vi "Event Handler.vi"(0 "uService Template in":refnum<class "Dummy.lvclass">, 5 "Event type":T1=enum."Message", 7 "Item Name":string, 9 "Data":variant, 11 "error in (no error)":errorcluster) -> (4 "uService Template out":refnum<class "Dummy.lvclass">, 15 "error out":errorcluster)   [LabVIEW 2020, in "Dummy.lvlib" / "Dummy.lvclass"]
doc: "This VI is the event handler of the uService: every time an event is triggered to the uService, this VI is called.\nNote: here you can access the Actor/Class data, but it will be the one coming out from Init. You cannot modify the values.\nThree different events are supported:\nI) Button Pressed: get called on a GUI button pressed. Item Name is the name (label) of the button, Data is empty.\nII) Shared Variable Updated: get called when a SV you subscribed to is updated. Item Name is the name of the SV, and Data is the value (note: you need to convert it to the proper type).\nIII) Message: get called every time a user event is generated using Send Message to Event Handler. The values of Item Name and Data are the one given to the Send Message to Event Handler.\nIV) Ready to launch?: this frame get called every time a new Run is initiated. Each uService is responsible of performing a self check before giving back the green light for the Run to start."
uses:
  Dummy.lvclass
  Dummy.lvclass/Dummy.ctl
  TALOS/TALOS_PPL.lvlibp/Father of all uServices/Father of all uServices/Father of all uServices.lvclass
  C:/LabVIEW Code/aegis-labview-code/TALOS/TALOS_PPL.lvlibp/Father of all uServices/Father of all uServices/Father of all uServices.lvclass
  TALOS/TALOS_PPL.lvlibp/Father of all uServices/Father of all uServices/Event Handler Items.ctl
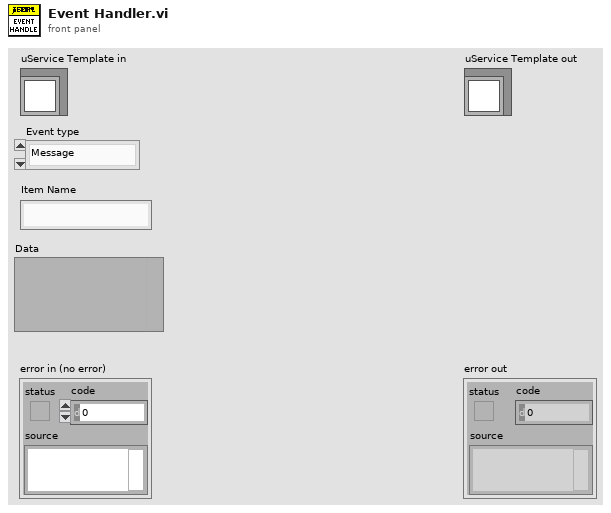
[diagram p1: front panel]
types:
  T1 = typedef "TALOS_PPL.lvlibp/Father of all uServices.lvlib/Father of all uServices.lvclass/Event Handler Items.ctl" = enum16{"Button Pressed", "Message", "Ready to launch?", "Safe Mode", "Start RUN", "Stop RUN"}
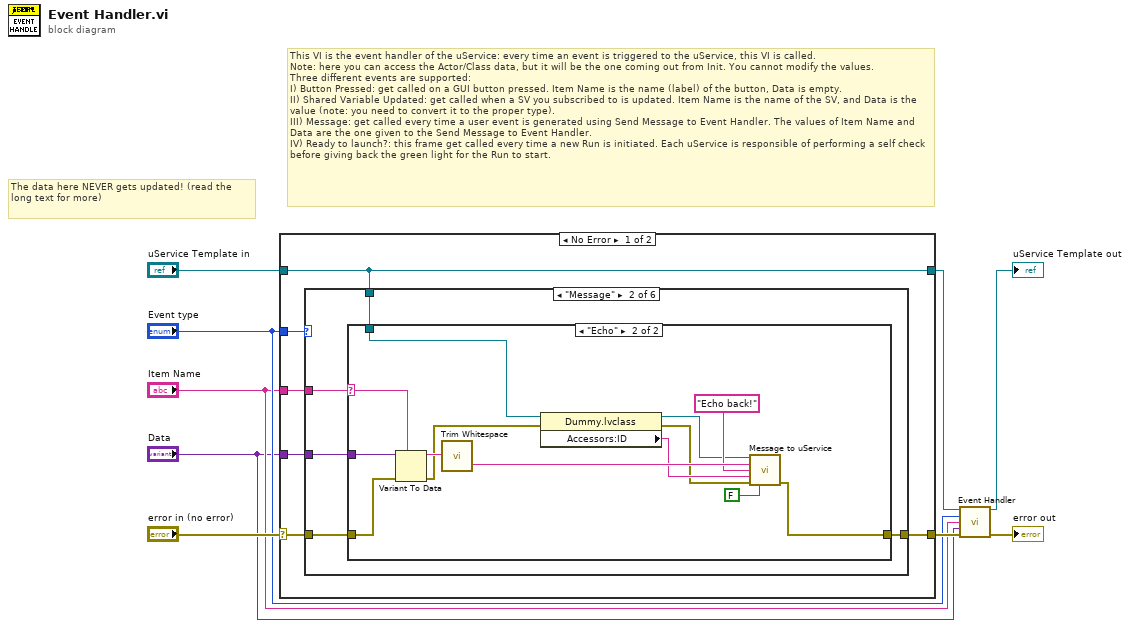
[diagram p0: block diagram]
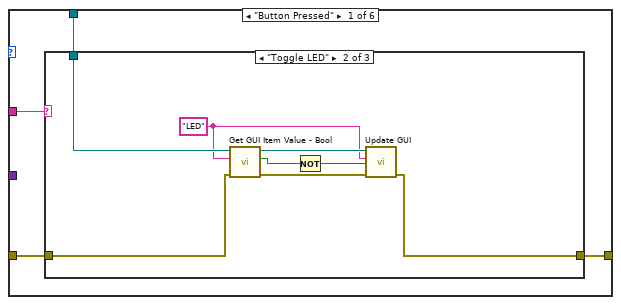
[diagram p2: hidden frame]
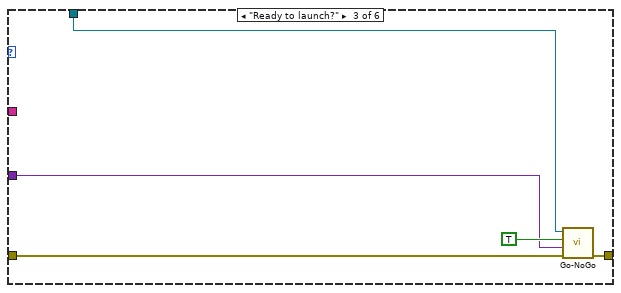
[diagram p6: hidden frame]
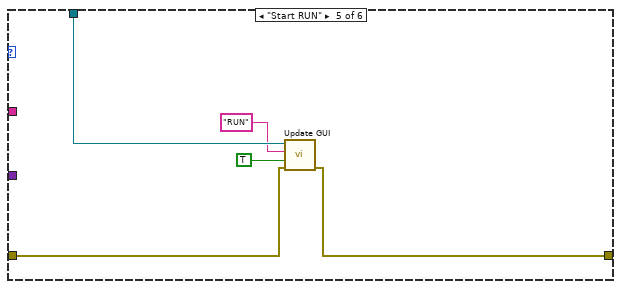
[diagram p8: hidden frame]
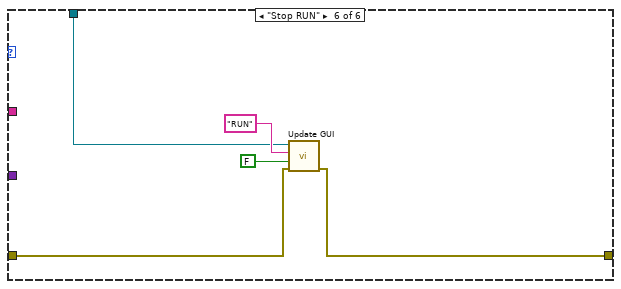
[diagram p9: hidden frame]
diagram:
  # "The data here NEVER gets updated! (read the long text for more)"
  # "This VI is the event handler of the uService: every time an event is triggered to the uService, this VI is called.\nNote: here you can access the Actor/Class data, but it will be the one coming out from Init. You cannot modify the values.\nThree different events are supported:\nI) Button Pressed: get called on a GUI button pressed. Item Name is the name (label) of the button, Data is empty.\nII) Shared Variable Updated: get called when a SV you subscribed to is updated. Item Name is the name of the SV, and Data is the value (note: you need to convert it to the proper type).\nIII) Message: get called every time a user event is generated using Send Message to Event Handler. The values of Item Name and Data are the one given to the Send Message to Event Handler.\nIV) Ready to launch?: this frame get called every time a new Run is initiated. Each uService is responsible of performing a self check before giving back the green light for the Run to start."
  n1 = case shown="No Error" "error in (no error)" {
    selector: "error in (no error)" -> [w13 w66]
    tunnel: [w14 w66] -> w7
    tunnel: [w12 w65] -> w4
    tunnel: "uService Template in" -> [w12 w65]
    tunnel: "Event type" -> [w15 _]
    tunnel: "Item Name" -> [w11 _]
    tunnel: "Data" -> [w10 _]
    frame No Error {
      n2 = case shown="\"Message\"" w15 {
        tunnel: [w19 w30 w52 w54 w56 w61] -> w14
        tunnel: w13 -> [w16 w34 w53 w54 w55 w60]
        tunnel: w11 -> [w17 w33 _ _ _ _]
        tunnel: w12 -> [w18 w31 w51 _ w59 w62]
        tunnel: w10 -> [_ w32 w49 _ _ _]
        frame "Button Pressed" {
          n3 = case shown="\"Toggle LED\"" w17 {
            tunnel: w16 -> [w20 w21 w29]
            tunnel: [w20 w22 w29] -> w19
            tunnel: w18 -> [_ w26 _]
            frame Default {
            }
            frame "Toggle LED" {
              w25 = "LED" ("FP Item Name")
              n4 = call "Get GUI Item Value - Bool.vi"("error in (no error)"=w21, "FP Item Name"=w25, "uService Template in"=w26) -> ("error out"=w28:errorcluster, "Value"=w24:bool, "uService Template out"=w27:refnum<class "Dummy.lvclass">)  [unwired: 6 in]
              n5 = Not(x=w24) -> (.not. x?=w23:bool)
              n6 = call "Update GUI.vi"("error in (no error)"=w28, "Data"=w23, "GUI Item Name"=w25, "uService Template in"=w27) -> ("error out"=w22:errorcluster)  [unwired: 6 in, 1 out]
            }
            frame "Test" {
            }
          }
        }
        frame "Message" {
          n7 = case shown="\"Echo\"" w33 {
            selector: w33 -> [_ w47]
            tunnel: w34 -> [w35 w39]
            tunnel: w32 -> [_ w48]
            tunnel: w31 -> [_ w40]
            tunnel: [w35 w43] -> w30
            frame Default {
            }
            frame "Echo" {
              n8 = Variant To Data(error in=w39, type=w47, Variant=w48) -> (data=w46:string, error out=w38:errorcluster)
              n9 = call <vilib>:"Trim Whitespace.vi"("string"=w46) -> ("trimmed string"=w45:string)  [unwired: 1 in]
              n10 = property class="Dummy.lvclass"(reference=w40, error in=w38) -> (reference out=w41:refnum<class "Dummy.lvclass">, error out=w36:errorcluster, "Accessors:ID"=w37:string)
              n11 = call "Message to uService.vi"("Father of all uServices in"=w41, "uService ID"=w45, "Message"="Echo back!", "Data"=w37, "error in (no error)"=w36, "Locale?"=FALSE) -> ("error out"=w43:errorcluster)  [unwired: 8 in, 1 out]
            }
          }
        }
        frame "Ready to launch?" {
          n12 = call-dynamic "Go-NoGo.vi"("error in (no error)"=w53, "Go-NoGo Data"=w49, "Go?"=TRUE, "Father of all uServices in"=w51) -> ("error out"=w52:errorcluster)  [unwired: 6 in, 1 out]
        }
        frame "Safe Mode" {
        }
        frame "Start RUN" {
          n13 = call "Update GUI.vi"("error in (no error)"=w55, "Data"=TRUE, "GUI Item Name"="RUN", "uService Template in"=w59) -> ("error out"=w56:errorcluster)  [unwired: 6 in, 1 out]
        }
        frame "Stop RUN" {
          n14 = call "Update GUI.vi"("error in (no error)"=w60, "Data"=FALSE, "GUI Item Name"="RUN", "uService Template in"=w62) -> ("error out"=w61:errorcluster)  [unwired: 6 in, 1 out]
        }
      }
    }
    frame Error {
    }
  }
  n15 = call-parent "Event Handler.vi"("uService Template in"=w4, "Event type"="Event type", "Item Name"="Item Name", "Data"="Data", "error in (no error)"=w7) -> ("uService Template out"=→"uService Template out":refnum<class "Dummy.lvclass">, "error out"=→"error out":errorcluster)  [unwired: 9 in]
